vi "wait for udp trigger.vi"(8 "error in (no error)":errorcluster) -> (0 "No error":errorcluster)   [LabVIEW 2020]
panel:
  out "connection ID":refnum<k16>
  out "Received Data":dbl(graph)
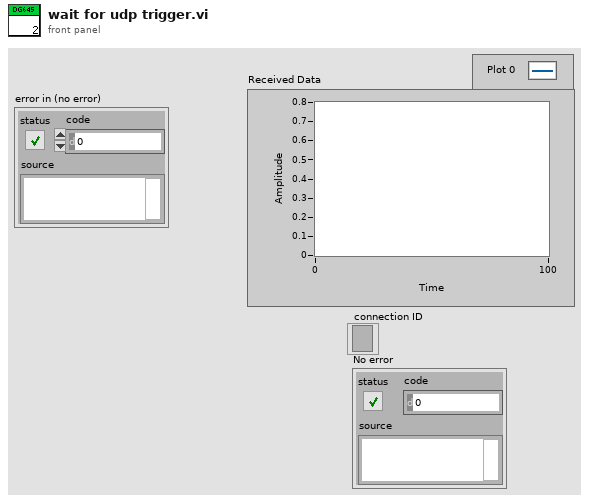
[diagram p1: front panel]
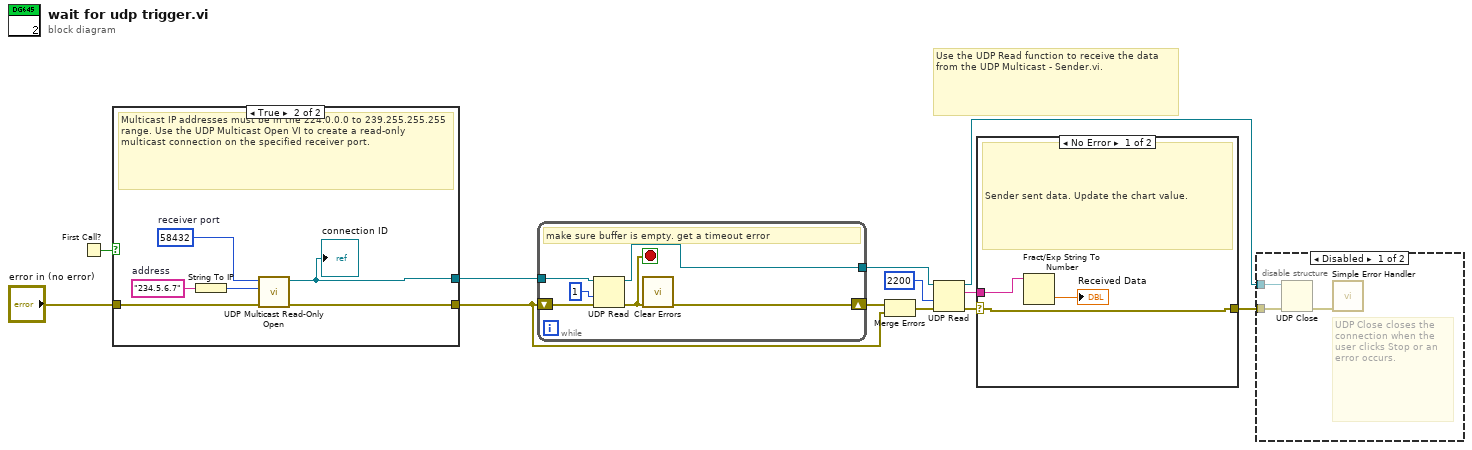
[diagram p0: block diagram]
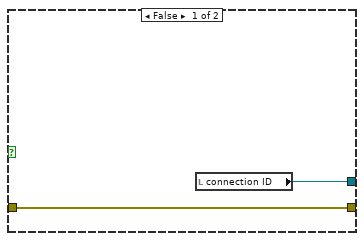
[diagram p2: hidden frame]
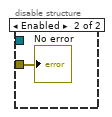
[diagram p3: hidden frame]
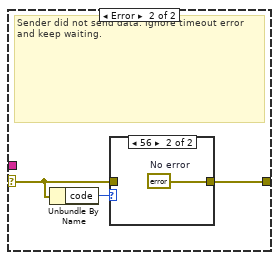
[diagram p4: hidden frame]
diagram:
  # "Use the UDP Read function to receive the data from the UDP Multicast - Sender.vi."
  n1 = First Call?() -> (First Call?: T/F=w11:bool)
  n2 = case shown="True" w11 {
    tunnel: [w14 w19] -> w4
    tunnel: [w13 w15] -> w2
    tunnel: "error in (no error)" -> [w14 w16]
    frame False {
      n3 = local read "connection ID"() -> (w13:refnum<k16>)
    }
    frame True {
      w18 = u16 58432  # receiver port
      w20 = "234.5.6.7"  # address
      # "Multicast IP addresses must be in the 224.0.0.0 to 239.255.255.255 range. Use the UDP Multicast Open VI to create a read-only multicast connection on the specified receiver port."
      n4 = String To IP(1:w20) -> (0:w17:u32)
      n5 = call "UDP Multicast Read-Only Open.vi"("error in (no error)"=w16, "multicast addr"=w17, "port"=w18) -> ("error out"=w19:errorcluster, "connection ID"=w15:refnum<k16>)  [unwired: 6 in, 1 out]
      "connection ID" <- w15
    }
  }
  n6 = while {
    shift-right: [w25] -> w5
    shift-left: w4 -> [w24]
    tunnel: w2 -> [w22]
    tunnel: [w21] -> w1
    stop <- w23 stop-if-true
    # "make sure buffer is empty. get a timeout error"
    n7 = UDP Read(connection ID=w22, timeout ms (25000)=1, 8:w24) -> (error out=w23:errorcluster, 3:w21:refnum<k16>)  [unwired: 4 out]
    n8 = call "Clear Errors.vi"("error in (no error)"=w23) -> ("error out"=w25:errorcluster)  [unwired: 5 in, 1 out]
  }
  n9 = Merge Errors(w5, w4) -> (w3:errorcluster)
  n10 = UDP Read(connection ID=w1, timeout ms (25000)=2200, 8:w3) -> (data out=w9:string, error out=w10:errorcluster, 3:w6:refnum<k16>)  [unwired: 3 out]
  n11 = case shown="No Error" w10 {
    selector: w10 -> [w28 w31]
    tunnel: w9 -> [w29 _]
    tunnel: [w28 w30] -> w7
    frame No Error {
      # "Sender sent data. Update the chart value."
      n12 = Fract/Exp String To Number(string=w29) -> (number=→"Received Data":dbl)  [unwired: 3 in, 1 out]
    }
    frame Error {
      # "Sender did not send data. Ignore timeout error and keep waiting."
      n13 = Unbundle By Name(w31) -> ("code"=w32:i32)
      n14 = case shown="56" w32 {
        tunnel: w31 -> [w33 _]
        tunnel: [w33 w34] -> w30
        frame Default {
        }
        frame 56 {
          w34 = errorcluster {"status"=FALSE, "code"=0, "source"=""}  # No error
        }
      }
    }
  }
  n15 = disable-structure shown="Disabled" {
    disable-tunnel: w6 -> [w37 _]
    disable-tunnel: w7 -> [w35 w38]
    frame Disabled {
      # "UDP Close closes the connection when the user clicks Stop or an error occurs."
      n16 = UDP Close(connection ID=w37, 8:w35) -> (error out=w36:errorcluster)  [unwired: 1 out]
      n17 = call "Simple Error Handler.vi"("error in (no error)"=w36) -> ()  [unwired: 1 in, 8 out]
    }
    frame Enabled {
      "No error" <- w38
    }
  }
